vi "Get ClientID List.vi"(8 "error in (no error)":errorcluster, 11 "Server in":refnum<class "Server.lvclass">) -> (0 "error out":errorcluster, 1 "Nb Connections":u32, 2 "ClientIDs":string[](array[string]), 3 "Server out":refnum<class "Server.lvclass">)   [LabVIEW 2013, in "MQTT Server.lvlib" / "Server.lvclass"]
uses:
  Server.lvclass
  Server.lvclass/Server.ctl
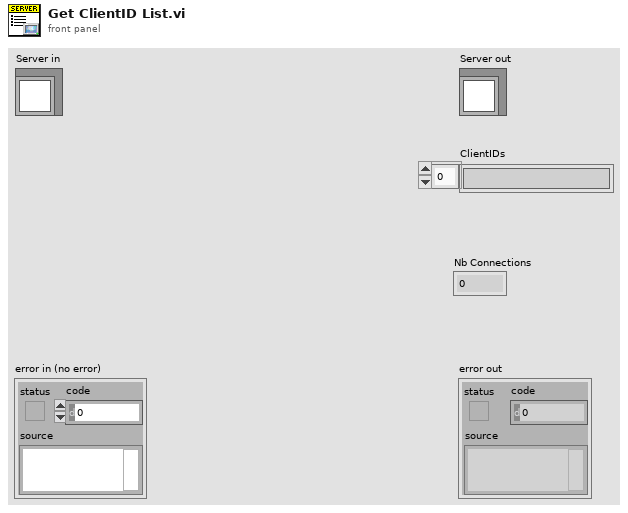
[diagram p1: front panel]
types:
  T1 = typedef "MQTT Server.lvlib/Server.lvclass/SessionRef -- cluster.ctl" = cluster{"ClientID":string, "SessionMailbox":refnum<queue>}
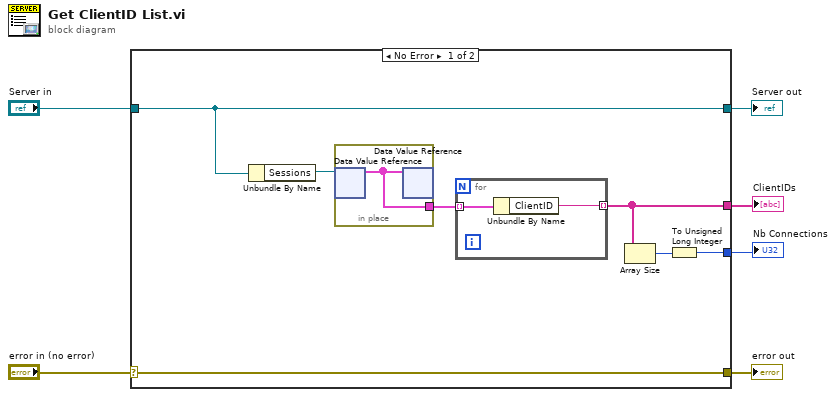
[diagram p0: block diagram]
diagram:
  n1 = case shown="No Error" "error in (no error)" {
    selector: "error in (no error)" -> [w13 w18]
    tunnel: [w13 w18] -> w5
    tunnel: [w12 w17] -> w3
    tunnel: "Server in" -> [w12 w17]
    tunnel: [w9 _] -> w2
    tunnel: [w7 _] -> w1
    frame No Error {
      n2 = Unbundle By Name(w12) -> ("Sessions"=w11:refnum<data-value>)
      n3 = in-place {
        in-place-border: [w16] -> w10
        n4 = in-place-dvr #1(w11) -> (w16:T1[])  [unwired: 1 out]
        n5 = in-place-dvr #1(w16) -> ()  [unwired: 2 out]
      }
      n6 = for {
        tunnel: w10 -> [w15] mode=indexing
        tunnel: [w14] -> w9 mode=indexing
        n7 = Unbundle By Name(w15) -> ("ClientID"=w14:string)
      }
      n8 = Array Size(array=w9) -> (size(s)=w8:i32)
      n9 = To Unsigned Long Integer(number=w8) -> (unsigned 32bit integer=w7:u32)
    }
    frame Error {
    }
  }
  "error out" <- w5
  "Server out" <- w3
  "ClientIDs" <- w2
  "Nb Connections" <- w1
